vi "Template Project Name--constant.vi"() -> (3 "Template Project Name":string)   [LabVIEW 2026]
doc: "This constant defines the name of the template project."
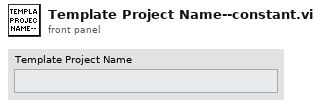
[diagram p1: front panel]
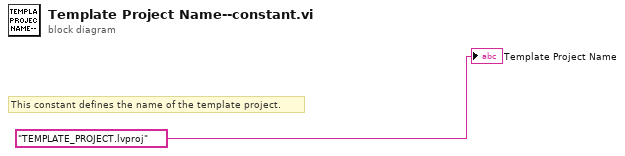
[diagram p0: block diagram]
diagram:
  # "This constant defines the name of the template project."
  "Template Project Name" <- "TEMPLATE_PROJECT.lvproj"
